vi "Iceoryx I64 Tag.vi"() -> (3 "CIF_CIPC_Chn_I64.lvclass":refnum<class "CIF_Iceoryx_Chn_I64.lvclass">)   [LabVIEW 2021, in "CIF_Iceoryx_Chn_I64.lvclass"]
uses:
  CIF_Iceoryx_Chn_I64.lvclass
  CIF_Iceoryx_Chn_I64.lvclass/CIF_Iceoryx_Chn_I64.ctl
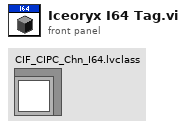
[diagram p1: front panel]
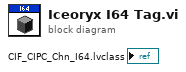
[diagram p0: block diagram]
diagram:
